vi "VI Tester Project API Open and Run All Tests.vi"(8 "error in":errorcluster, 11 "Object":T1) -> (0 "error out":errorcluster)   [LabVIEW 2013]
uses:
  VITester Project Item Ref.ctl
  VI Tester Project API Method Selector - Enum.ctl
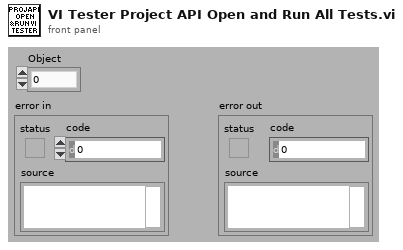
[diagram p1: front panel]
types:
  T1 = typedef "VITester Project Item Ref.ctl" = u64
  T2 = typedef "VI Tester Project API Method Selector - Enum.ctl" = enum16{"Open VI Tester", "Run All Tests", "Create New TestCase", "Create New TestSuite"}
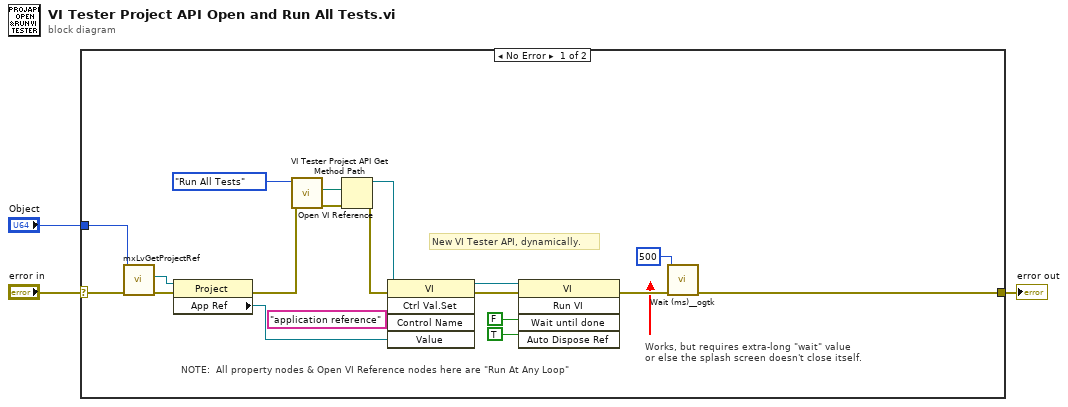
[diagram p0: block diagram]
diagram:
  n1 = case shown="No Error" "error in" {
    selector: "error in" -> [w8 w23]
    tunnel: [w22 w23] -> w3
    tunnel: "Object" -> [w20 _]
    frame No Error {
      # "Works, but requires extra-long \"wait\" value\nor else the splash screen doesn't close itself."
      # "NOTE:  All property nodes & Open VI Reference nodes here are \"Run At Any Loop\""
      # "New VI Tester API, dynamically."
      n2 = call <resource>:"mxLvGetProjectRef.vi"("error in"=w8, "Item"=w20) -> ("error out"=w10:errorcluster, "Project Refnum"=w11:refnum<vi>)  [unwired: 7 in, 1 out]
      n3 = property class="Project"(reference=w11, error in=w10) -> (error out=w6:errorcluster, "App Ref"=w9:refnum<vi>)  [unwired: 1 out]
      n4 = call "VI Tester Project API Get Method Path.vi"("error in (no error)"=w6, "Project API Method"=VI_Tester_Project_API_Method_Selector_-_Enum."Run All Tests") -> ("error out"=w5:errorcluster, "Path to VI Tester Project API Proxy VI"=w21:path)  [unwired: 8 in]
      n5 = Open VI Reference(vi path=w21, error in (no error)=w5) -> (vi reference=w14:refnum<vi>, error out=w16:errorcluster)  [unwired: 4 in]
      n6 = invoke class="VI" method="Ctrl Val.Set"(reference=w14, error in=w16, "Control Name"="application reference", "Value"=w9) -> (reference out=w13:refnum<vi>, error out=w15:errorcluster)  [unwired: 1 in, 3 out]
      n7 = invoke class="VI" method="Run VI"(reference=w13, error in=w15, "Wait until done"=FALSE ("Wait Until Done"), "Auto Dispose Ref"=TRUE ("Auto Dispose Reference")) -> (error out=w17:errorcluster)  [unwired: 1 in, 4 out]
      n8 = call <userlib>:"Wait (ms)__ogtk.vi"("error in (no error)"=w17, "milliseconds to wait"=u32 500) -> ("error out"=w22:errorcluster)  [unwired: 8 in, 1 out]
    }
    frame Error {
    }
  }
  "error out" <- w3
